vi "Replace Output Type Cluster Constant by Type Definition.vi"(8 "error in":errorcluster, 11 "Virtual Instrument in":refnum<class "Virtual Instrument.lvclass">) -> (0 "error out":errorcluster, 3 "Virtual Instrument out":refnum<class "Virtual Instrument.lvclass">)   [LabVIEW 2026, in "Virtual Instrument.lvclass"]
doc: "Replace the cluster constant that defines the datatype of the output of the python node by the corresponding type definition."
uses:
  Virtual Instrument.lvclass
  <vilib>/Utility/traverseref.llb/TRef TravTarget.ctl
  Type Definitions/Parameter Mode--enum.ctl
  Virtual Instrument.lvclass/Virtual Instrument.ctl
  LabVIEW File/LabVIEW File.lvclass/LabVIEW File.ctl
  LabVIEW File/Read VI Reference.vi
  LabVIEW File/Read Name.vi
  <userlib>/_OpenG.lib/file/file.llb/File Exists - Scalar__ogtk.vi
  <userlib>/_OpenG.lib/file/file.llb/openg_file.lvlib
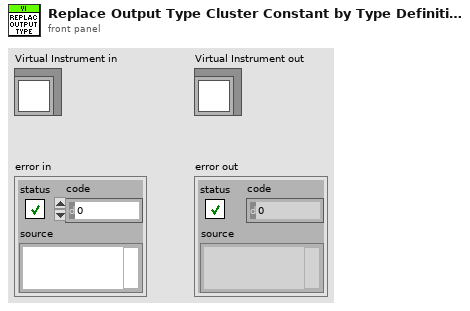
[diagram p1: front panel]
types:
  T1 = typedef "Parameter Mode--enum.ctl" = enum16{"Input", "Output"}
  T2 = typedef "TRef TravTarget.ctl" = enum16{"FP", "BD", "Other"}
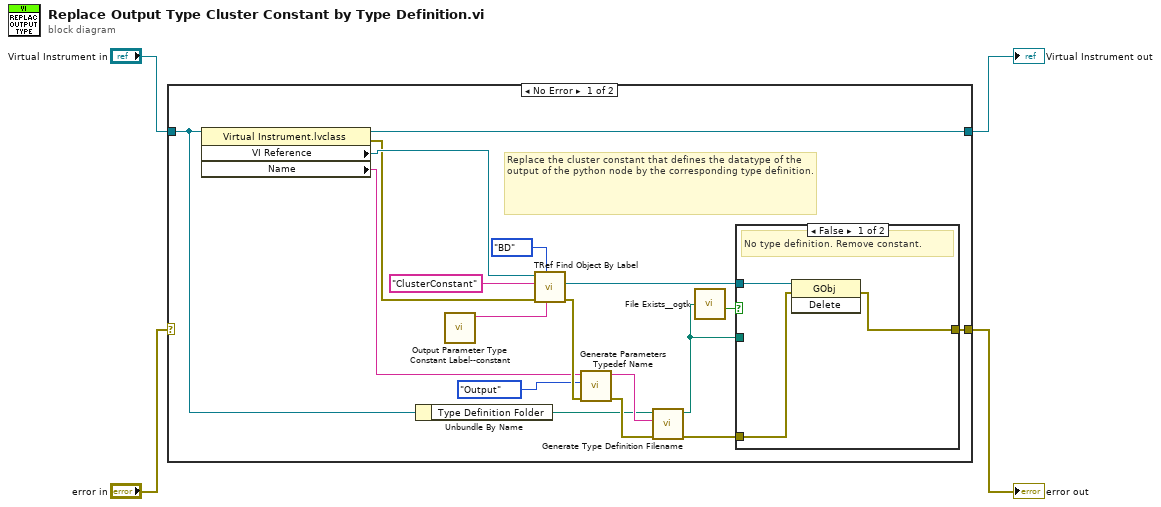
[diagram p0: block diagram]
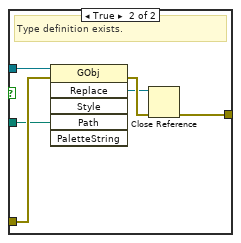
[diagram p2: hidden frame]
diagram:
  n1 = case shown="No Error" "error in" {
    selector: "error in" -> [_ w33]
    tunnel: [w19 w33] -> w3
    tunnel: [w8 w32] -> w1
    tunnel: "Virtual Instrument in" -> [w9 w32]
    frame No Error {
      # "Replace the cluster constant that defines the datatype of the output of the python node by the corresponding type definition."
      n2 = property class="Virtual Instrument.lvclass"(reference=w9) -> (reference out=w8:refnum<class "Virtual Instrument.lvclass">, error out=w6:errorcluster, "VI Reference"=w7:refnum<vi>, "Name"=w5:string)  [unwired: 1 in]
      n3 = Unbundle By Name(w9) -> ("Type Definition Folder"=w14:path)
      n4 = call "Output Parameter Type Constant Label--constant.vi"() -> ("Output Parameter Type Constant Label"=w13:string)  [unwired: 11 in]
      n5 = call <vilib>:"TRef Find Object By Label.vi"("Label"=w13, "Traverse Target"=TRef_TravTarget."BD", "error in (no error)"=w6, "Class Name"="ClusterConstant", "VI Ref"=w7) -> ("error out"=w22:errorcluster, "Found Obj Ref"=w16:refnum<vi>)  [unwired: 3 in, 2 out]
      n6 = call "Generate Parameters Typedef Name.vi"("error in"=w22, "Parameter Mode"=Parameter_Mode--enum."Output", "VI Name"=w5) -> ("error out"=w21:errorcluster, "Type Definition Name"=w15:string)  [unwired: 7 in]
      n7 = call "Generate Type Definition Filename.vi"("error in"=w21, "Name"=w15, "Path"=w14) -> ("error out"=w20:errorcluster, "Typedef Path"=w11:path)  [unwired: 7 in]
      n8 = call-poly <userlib>:"File Exists__ogtk.vi"("file path"=w11) -> ("exists"=w10:bool)  [unwired: 6 in, 1 out]
      n9 = case shown="False" w10 {
        tunnel: w20 -> [w24 w31]
        tunnel: [w25 w29] -> w19
        tunnel: w16 -> [w23 w28]
        tunnel: w11 -> [_ w27]
        frame False {
          # "No type definition. Remove constant."
          n10 = invoke class="GObj" method="Delete"(reference=w23, error in=w24) -> (error out=w25:errorcluster)  [unwired: 1 in, 2 out]
        }
        frame True {
          # "Type definition exists."
          n11 = invoke class="GObj" method="Replace"(reference=w28, error in=w31, "Path"=w27) -> (error out=w30:errorcluster, "Replace"=w26:refnum<vi>)  [unwired: 3 in, 4 out]
          n12 = Close Reference(reference=w26, error in (no error)=w30) -> (error out=w29:errorcluster)
        }
      }
    }
    frame Error {
    }
  }
  "error out" <- w3
  "Virtual Instrument out" <- w1
